vi "Init Msg Input.vi"(6 "Teller":refnum<class "Teller.lvclass">, 9 "Parent Stopped":bool, 10 "Safe Stop":bool=TRUE) -> (2 "Msg Input":refnum<class "Msg Input.lvclass">)   [LabVIEW 2020, in "jettl.lvlib" / "Stop jettl Msg.lvlib" / "Stop Msg Input.lvlib"]
uses:
  Stop Msg Input.lvlib
  Msg Input/Msg Input.lvclass
  Teller/Teller.lvclass
  Stop Msg Input/Stop Msg Input.lvclass/Stop Msg Input.ctl
  Stop Msg Input/Stop Msg Input.lvclass
  C:/git/jettl/src/jettl/jettl/Msg Input/Msg Input.lvclass
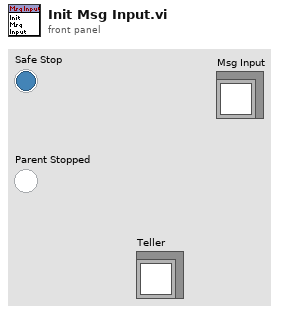
[diagram p1: front panel]
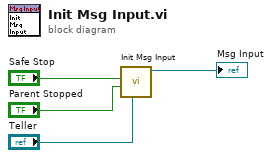
[diagram p0: block diagram]
diagram:
  n1 = call "Init Msg Input.vi"("Teller"="Teller", "Parent Stopped"="Parent Stopped", "Safe Stop"="Safe Stop") -> ("Stop Msg Input out"=→"Msg Input":refnum<class "Stop Msg Input.lvclass">)  [unwired: 8 in]
